vi "Read IExporter.vi"(10 "Path":path, 11 "CDependencyInspection in":refnum<class "CDependencyInspection.lvclass">) -> (0 "error out":errorcluster, 1 "IExporter":refnum<class "IExporter.lvclass">, 3 "CDependencyInspection out":refnum<class "CDependencyInspection.lvclass">)   [LabVIEW 2020, in "DependencyInspection.lvlib" / "CDependencyInspection.lvclass"]
uses:
  CDependencyInspection.lvclass
  ExtensionInterfaces/IExporter/IExporter.lvclass
  CDependencyInspection.lvclass/CDependencyInspection.ctl
  74d57e81-e5c7-405e-903f-d7f88fe582b6.vi
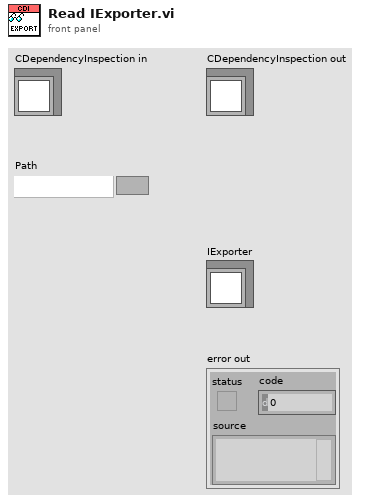
[diagram p1: front panel]
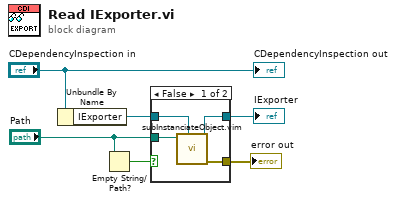
[diagram p0: block diagram]
diagram:
  n1 = Unbundle By Name("CDependencyInspection in") -> ("IExporter"=w3:refnum<class "IExporter.lvclass">)
  n2 = Empty String/Path?(string/path="Path") -> (empty?=w4:bool)
  n3 = case shown="False" w4 {
    tunnel: "Path" -> [w10 _]
    tunnel: w3 -> [w9 w11]
    tunnel: [w8 w11] -> w2
    tunnel: [w7 _] -> w1
    frame False {
      n4 = call "subInstanciateObject.vim"("Target object"=w9, "Class path"=w10) -> ("error out"=w7:errorcluster, "Object"=w8:refnum<class "IExporter.lvclass">)  [unwired: 8 in]
    }
    frame True {
    }
  }
  "IExporter" <- w2
  "error out" <- w1
  "CDependencyInspection out" <- "CDependencyInspection in"
